vi "Connect.vi"(8 "error in (no error)":errorcluster, 10 "Connection":T1 {"Custom Data" format="%.0x"}, 11 "CIFTag in":refnum<class "CIF_CIPC_Chn.lvclass">) -> (0 "error out":errorcluster, 3 "CIFTag out":refnum<class "CIF_CIPC_Chn.lvclass">)   [LabVIEW 2021, in "CIF_CIPC_Chn.lvclass"]
uses:
  CIF_CIPC_Chn.lvclass
  C:/Program Files/National Instruments/LabVIEW 2021/vi.lib/CIF Foundation/CIF Channels Core/CIFChannels/CIFChannels.lvclass
  <vilib>/CIF Foundation/CIF Channels Core/ChannelCommon/typedef/New FIFO Instance Response.ctl
  <vilib>/CIF Foundation/CIF Channels Core/CIFChannels/CIFChannels.lvclass/CIFChannels.ctl
  CIF_CIPC_Chn.lvclass/CIF_CIPC_Chn.ctl
  <vilib>/CIF Foundation/CIF Channels Core/ChannelCommon/typedef/Channel State.ctl
  <vilib>/CIF Foundation/CIF Channels Core/CIFChannels/Accessors/Read Direction.vi
  <vilib>/CIF Foundation/CIF Channels Core/CIFChannels/CIFChannels.lvclass
  <vilib>/CIF Foundation/CIF Channels Core/ChannelCommon/ChannelCommon.lvlib
  <vilib>/CIF Foundation/CIF CIPC/CIF_NI_CIPC.lvlib
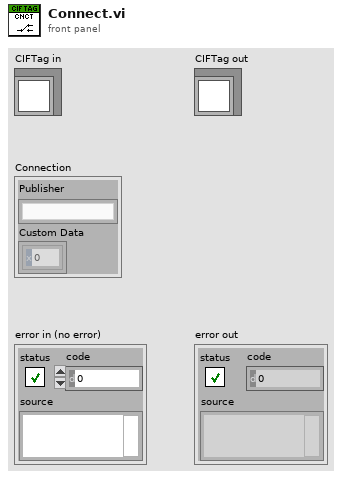
[diagram p1: front panel]
types:
  T1 = typedef "ChannelCommon.lvlib/New FIFO Instance Response.ctl" = cluster{"Publisher":string, "Custom Data":u8[]}
  T2 = typedef "ChannelCommon.lvlib/Channel State.ctl" = enum8{"Creating", "Disconnected", "Connecting", "Connected", "Destroyed"}
  T3 = typedef "ChannelCommon.lvlib/Direction.ctl" = enum8{"Publisher", "Subscriber"}
  T4 = typedef "CIF_CIPC_Chn.lvclass/Buffer Configuration Data.ctl" = cluster{"Total Size":u32, "Read Size":u32, "Read Offset":u32, "CIPC BP References":T5, "CIPC Backpressure Names":T6, "Override CIPC Name":string, "Encoder Data":string}
  T5 = typedef "CIF_NI_CIPC.lvlib/Backpressure References.ctl" = cluster{"CIPC Reference":u64, "CIPC BP Reference":u64}
  T6 = typedef "CIF_NI_CIPC.lvlib/Backpressure Names.ctl" = cluster{"CIPC Name":string, "CIPC BP Name":string}
  T7 = typedef "CIF_NI_CIPC.lvlib/Encoder Info.ctl" = cluster{"Name":string, "Version":i32, "Data":string}
  T8 = typedef "NI_Data Type.lvlib/Data Type.ctl" = enum8{"Invalid Type", "Void", "I8", "I16", "I32", "I64", "U8", "U16", "U32", "U64", "Single Float", "Double Float", "Extended Float", "Single Complex", "Double Complex", "Extended Complex", "Enum U8", "Enum U16", "Enum U32", "Enum U64", "Single Float With Unit", "Double Float With Unit", "Extended Float With Unit", "Single Complex with Unit", "Double Complex with Unit", "Extended Complex with Unit", "Boolean", "String", "Path", "Picture", "Tag", "Array", "Cluster", "Variant", "LV Variant", "Waveform", "Timestamp", "Digital Waveform", "Digital Data", "ExpressData", "Refnum", "External Data", "VI", "Poly VI", "LabVIEW Class Instance", "Fixed Point", "Set Collection", "Map Collection"}
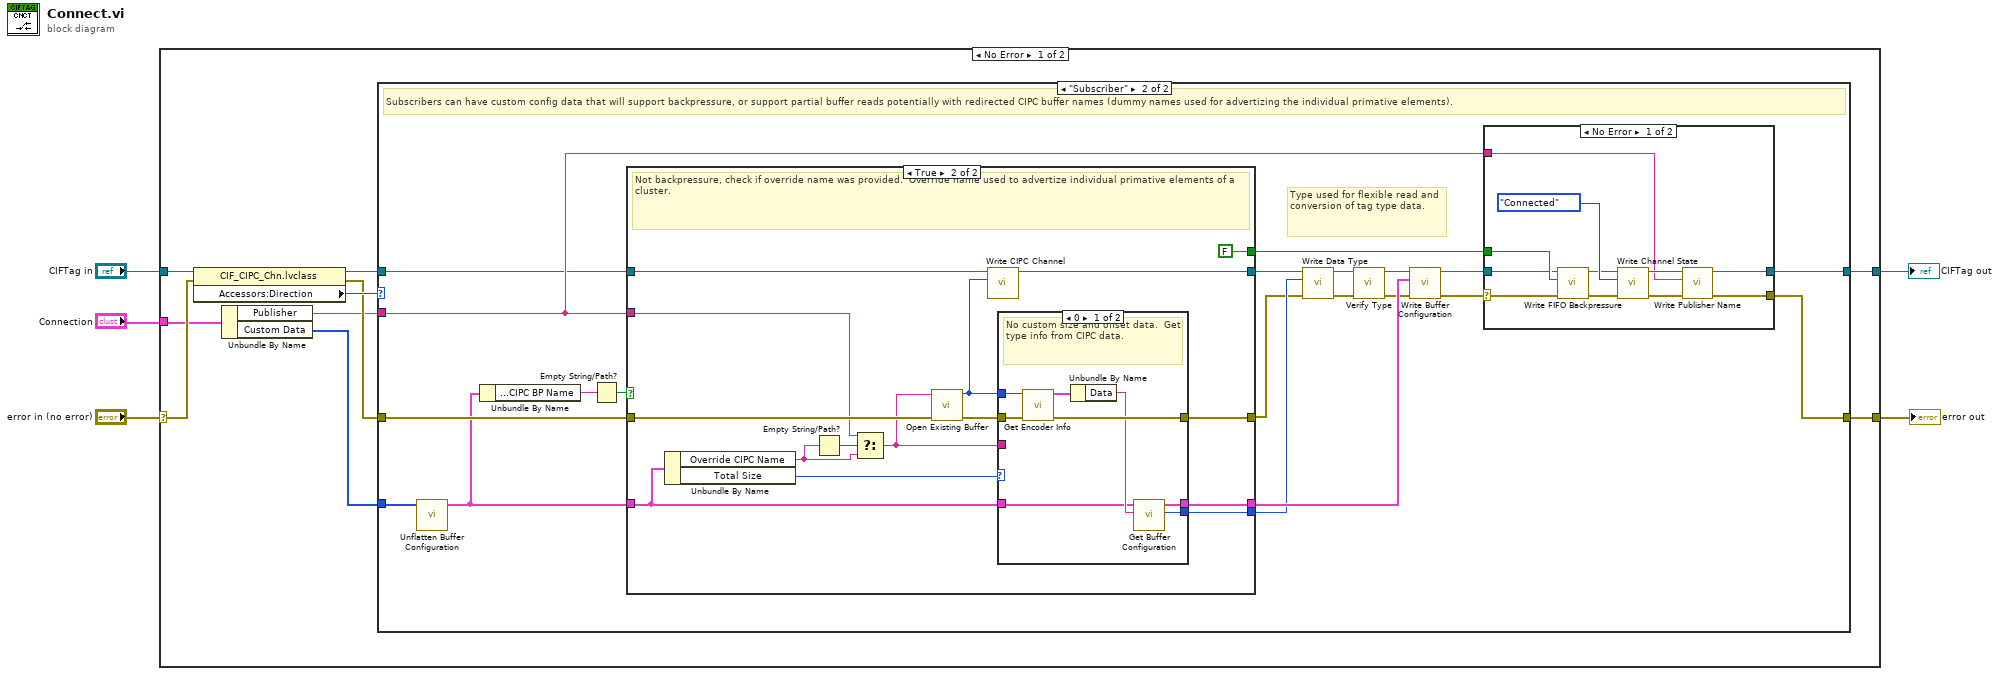
[diagram p0: block diagram]
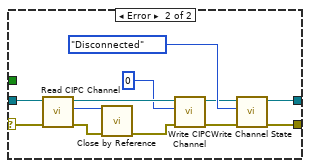
[diagram p3: hidden frame]
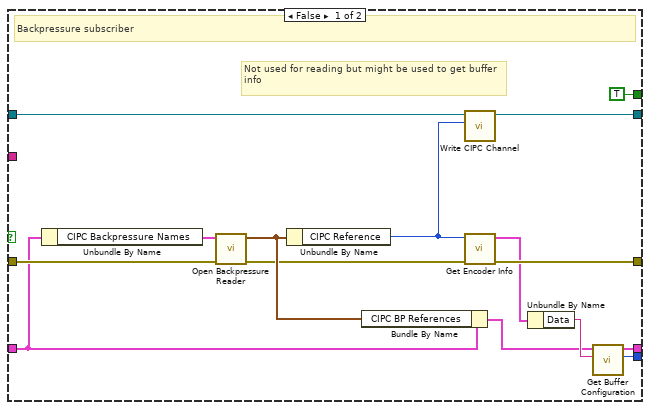
[diagram p4: hidden frame]
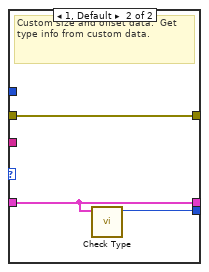
[diagram p5: hidden frame]
diagram:
  n1 = case shown="No Error" "error in (no error)" {
    selector: "error in (no error)" -> [w14 w103]
    tunnel: [w9 w103] -> w4
    tunnel: [w11 w102] -> w2
    tunnel: "CIFTag in" -> [w15 w102]
    tunnel: "Connection" -> [w8 _]
    frame No Error {
      n2 = property class="CIF_CIPC_Chn.lvclass"(reference=w15, error in=w14) -> (reference out=w13:refnum<class "CIF_CIPC_Chn.lvclass">, error out=w10:errorcluster, "Accessors:Direction"=w12:T3)
      n3 = Unbundle By Name(w8) -> ("Publisher"=w7:string, "Custom Data"=w6:u8[])
      n4 = case shown="\"Subscriber\"" w12 {
        tunnel: w13 -> [w17 w29]
        tunnel: [w17 w25] -> w11
        tunnel: w10 -> [w16 w37]
        tunnel: w7 -> [_ w30]
        tunnel: [w16 w24] -> w9
        tunnel: w6 -> [_ w32]
        frame "Publisher" {
          # "No connection step needed for publishers"
        }
        frame "Subscriber" {
          # "Type used for flexible read and conversion of tag type data."
          # "Subscribers can have custom config data that will support backpressure, or support partial buffer reads potentially with redirected CIPC buffer names (dummy names used for advertizing the individual primative elements)."
          n5 = call "Unflatten Buffer Configuration.vi"("Flattened Configuration"=w32) -> ("Buffer Configuration"=w31:T4)  [unwired: 10 in]
          n6 = Unbundle By Name(w31) -> ("CIPC Backpressure Names.CIPC BP Name"=w27:string)
          n7 = Empty String/Path?(string/path=w27) -> (empty?=w26:bool)
          n8 = case shown="True" w26 {
            tunnel: w37 -> [w66 w90]
            tunnel: [w74 w89] -> w36
            tunnel: [w73 w88] -> w35
            tunnel: w31 -> [w65 w83]
            tunnel: w30 -> [_ w82]
            tunnel: w29 -> [w70 w80]
            tunnel: [w69 w79] -> w23
            tunnel: [w75 w77] -> w22
            tunnel: [TRUE ("Backpressure") FALSE ("Backpressure")] -> w28
            frame False {
              # "Not used for reading but might be used to get buffer info"
              # "Backpressure subscriber"
              n9 = Unbundle By Name(w65) -> ("CIPC Backpressure Names"=w67:T6)
              n10 = call <vilib>:"Open Backpressure Reader.vi"("error in (no error)"=w66, "CIPC Backpressure Names"=w67) -> ("error out"=w62:errorcluster, "CIPC BP References"=w64:T5)  [unwired: 8 in]
              n11 = Unbundle By Name(w64) -> ("CIPC Reference"=w61:u64)
              n12 = Bundle By Name(cluster=w65, "CIPC BP References"=w64) -> (w63:T4)
              n13 = call "Write CIPC Channel.vi"("CIF Channel"=w61, "CIFTag in"=w70) -> ("CIFTag out"=w69:refnum<class "CIF_CIPC_Chn.lvclass">)  [unwired: 8 in, 1 out]
              n14 = call <vilib>:"Get Encoder Info.vi"("error in (no error)"=w62, "CIPC Reference"=w61) -> ("error out"=w75:errorcluster, "Encoder Info"=w68:T7)  [unwired: 8 in]
              n15 = Unbundle By Name(w68) -> ("Data"=w72:string)
              n16 = call "Get Buffer Configuration.vi"("Encoder Data Description"=w72, "Buffer Configuration in"=w63) -> ("Type"=w73:T8, "Buffer Configuration out"=w74:T4)  [unwired: 8 in]
            }
            frame True {
              # "Not backpressure, check if override name was provided.  Override name used to advertize individual primative elements of a cluster."
              n17 = Unbundle By Name(w83) -> ("Override CIPC Name"=w86:string, "Total Size"=w85:u32)
              n18 = Empty String/Path?(string/path=w86) -> (empty?=w87:bool)
              n19 = Select(t=w82, s=w87, f=w86) -> (s? t:f=w84:string)
              n20 = call <vilib>:"Open Existing Buffer.vi"("error in (no error)"=w90, "buffer_name"=w84) -> ("error out"=w78:errorcluster, "CIPC Reference"=w81:u64)  [unwired: 8 in]
              n21 = call "Write CIPC Channel.vi"("CIF Channel"=w81, "CIFTag in"=w80) -> ("CIFTag out"=w79:refnum<class "CIF_CIPC_Chn.lvclass">)  [unwired: 8 in, 1 out]
              n22 = case shown="0" w85 {
                tunnel: [w96 w100] -> w89
                tunnel: w81 -> [w98 _]
                tunnel: [w95 w101] -> w88
                tunnel: w83 -> [w91 w100]
                tunnel: w84 -> [_ _]
                tunnel: w78 -> [w94 w99]
                tunnel: [w93 w99] -> w77
                frame 0 {
                  # "No custom size and offset data.  Get type info from CIPC data."
                  n23 = call <vilib>:"Get Encoder Info.vi"("error in (no error)"=w94, "CIPC Reference"=w98) -> ("error out"=w93:errorcluster, "Encoder Info"=w97:T7)  [unwired: 8 in]
                  n24 = Unbundle By Name(w97) -> ("Data"=w92:string)
                  n25 = call "Get Buffer Configuration.vi"("Encoder Data Description"=w92, "Buffer Configuration in"=w91) -> ("Type"=w95:T8, "Buffer Configuration out"=w96:T4)  [unwired: 8 in]
                }
                frame 1, Default {
                  # "Custom size and offset data.  Get type info from custom data."
                  n26 = call "Check Type.vi"("Buffer Configuration"=w100) -> ("Type"=w101:T8)  [unwired: 10 in]
                }
              }
            }
          }
          n27 = call "Write Data Type.vi"("error in (no error)"=w22, "Type Enum"=w35, "CIF_CIPC_Chn in"=w23) -> ("error out"=w33:errorcluster, "CIF_CIPC_Chn out"=w34:refnum<class "CIF_CIPC_Chn.lvclass">)  [unwired: 7 in]
          n28 = call-dynamic "Verify Type.vi"("error in (no error)"=w33, "CIF_CIPC_Chn in"=w34) -> ("error out"=w20:errorcluster, "CIF_CIPC_Chn out"=w21:refnum<class "CIF_CIPC_Chn.lvclass">)  [unwired: 8 in]
          n29 = call "Write Buffer Configuration.vi"("error in (no error)"=w20, "Buffer Configuration"=w36, "CIF_CIPC_Chn in"=w21) -> ("error out"=w19:errorcluster, "CIF_CIPC_Chn out"=w18:refnum<class "CIF_CIPC_Chn.lvclass">)  [unwired: 7 in]
          n30 = case shown="No Error" w19 {
            selector: w19 -> [w38 w56]
            tunnel: w30 -> [w45 _]
            tunnel: w28 -> [w42 _]
            tunnel: w18 -> [w41 w57]
            tunnel: [w40 w59] -> w25
            tunnel: [w39 w58] -> w24
            frame No Error {
              n31 = call <vilib>:"Write FIFO Backpressure.vi"("error in (no error)"=w38, "Backpressure"=w42, "CIFChannels in"=w41) -> ("error out"=w44:errorcluster, "CIFChannels out"=w43:refnum<class "CIF_CIPC_Chn.lvclass">)  [unwired: 7 in]
              n32 = call <vilib>:"Write Channel State.vi"("error in (no error)"=w44, "Channel State"=Channel_State."Connected", "CIFChannels in"=w43) -> ("error out"=w46:errorcluster, "CIFChannels out"=w47:refnum<class "CIF_CIPC_Chn.lvclass">)  [unwired: 7 in]
              n33 = call <vilib>:"Write Publisher Name.vi"("error in (no error)"=w46, "Publisher Name"=w45, "CIFChannels in"=w47) -> ("error out"=w39:errorcluster, "CIFChannels out"=w40:refnum<class "CIF_CIPC_Chn.lvclass">)  [unwired: 7 in]
            }
            frame Error {
              n34 = call "Read CIPC Channel.vi"("error in (no error)"=w56, "CIFTag in"=w57) -> ("error out"=w54:errorcluster, "CIPC Channel"=w55:u64, "CIFTag out"=w53:refnum<class "CIF_CIPC_Chn.lvclass">)  [unwired: 7 in]
              n35 = call <vilib>:"Close by Reference.vi"("error in (no error)"=w54, "CIPC Reference"=w55) -> ("error out"=w51:errorcluster)  [unwired: 9 in]
              n36 = call "Write CIPC Channel.vi"("error in (no error)"=w51, "CIF Channel"=u64 0, "CIFTag in"=w53) -> ("error out"=w49:errorcluster, "CIFTag out"=w50:refnum<class "CIF_CIPC_Chn.lvclass">)  [unwired: 7 in]
              n37 = call <vilib>:"Write Channel State.vi"("error in (no error)"=w49, "Channel State"=Channel_State."Disconnected", "CIFChannels in"=w50) -> ("error out"=w58:errorcluster, "CIFChannels out"=w59:refnum<class "CIF_CIPC_Chn.lvclass">)  [unwired: 7 in]
            }
          }
        }
      }
    }
    frame Error {
    }
  }
  "error out" <- w4
  "CIFTag out" <- w2
